vi "Test Serialize Arrays.vi"(8 "error in (no error)":errorcluster) -> (0 "error out":errorcluster)   [LabVIEW 2013]
uses:
  src/Serializer/JSON Serializer/JSON Serializer.lvclass
  <vilib>/addons/_JKI Toolkits/Caraya/classes/Test/Test.lvclass
  <vilib>/addons/_JKI Toolkits/Caraya/classes/Assert/Assert.lvclass
  src/JKI JSON Serialization.lvlib
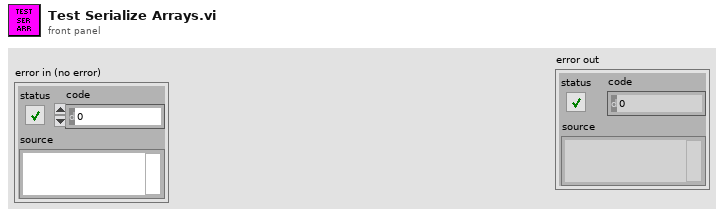
[diagram p1: front panel]
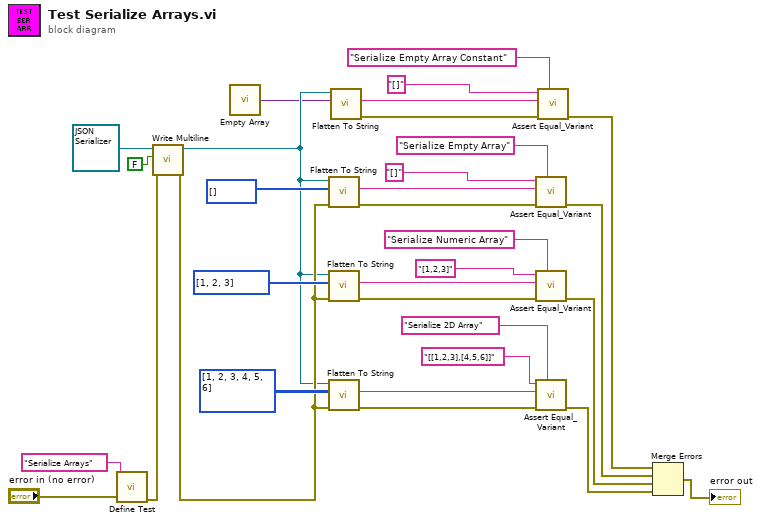
[diagram p0: block diagram]
diagram:
  n1 = call <vilib>:"Define Test.vi"("error in (no error)"="error in (no error)", "Label (VI Title)"="Serialize Arrays") -> ("error out"=w15:errorcluster)  [unwired: 9 in]
  n2 = call-dynamic "Write Multiline.vi"("error in (no error)"=w15, "Multiline"=FALSE, "JSON Serializer in"=refnum<class "JSON Serializer.lvclass"> refnum ("JKI JSON Serialization.lvlib:JSON Serializer.lvclass")) -> ("error out"=w12:errorcluster, "JSON Serializer out"=w3:refnum<class "JSON Serializer.lvclass">)  [unwired: 7 in]
  n3 = call "Empty Array.vi"() -> ("Empty Cluster"=w1:variant)
  n4 = call-dynamic "Flatten To String.vi"("error in (no error)"=w12, "Variant"=i32[] [], "JSON Serializer in"=w3) -> ("error out"=w27:errorcluster, "String"=w26:string)  [unwired: 6 in, 1 out]
  n5 = call-dynamic "Flatten To String.vi"("error in (no error)"=w12, "Variant"=i32[] [1, 2, 3], "JSON Serializer in"=w3) -> ("error out"=w31:errorcluster, "String"=w30:string)  [unwired: 6 in, 1 out]
  n6 = call-dynamic "Flatten To String.vi"("error in (no error)"=w12, "Variant"=i32[][] [[1, 2, 3], [4, 5, 6]], "JSON Serializer in"=w3) -> ("error out"=w8:errorcluster, "String"=w9:string)  [unwired: 6 in, 1 out]
  n7 = call-dynamic "Flatten To String.vi"("Variant"=w1, "JSON Serializer in"=w3) -> ("error out"=w7:errorcluster, "String"=w6:string)  [unwired: 7 in, 1 out]
  n8 = call <vilib>:"Assert Equal_Variant.vi"("Label"="Serialize Empty Array", "error in (no error)"=w27, "Y"=w26, "X"="[]") -> ("error out"=w20:errorcluster)  [unwired: 7 in]
  n9 = call <vilib>:"Assert Equal_Variant.vi"("Label"="Serialize Numeric Array", "error in (no error)"=w31, "Y"=w30, "X"="[1,2,3]") -> ("error out"=w21:errorcluster)  [unwired: 7 in]
  n10 = call <vilib>:"Assert Equal_Variant.vi"("Label"="Serialize 2D Array", "error in (no error)"=w8, "Y"=w9, "X"="[[1,2,3],[4,5,6]]") -> ("error out"=w22:errorcluster)  [unwired: 7 in]
  n11 = call <vilib>:"Assert Equal_Variant.vi"("Label"="Serialize Empty Array Constant", "error in (no error)"=w7, "Y"=w6, "X"="[]") -> ("error out"=w2:errorcluster)  [unwired: 7 in]
  n12 = Merge Errors(w2, w20, w21, w22) -> (→"error out":errorcluster)
